vi "WLAN_SNR_LTF.vi"(11 "LTF Corrected":cdb[](array[numeric])) -> (0 "SNR Valid?":bool, 1 "Noise Power":dbl, 2 "Signal Power":dbl, 3 "SNR dB":dbl)   [LabVIEW 2022 SP3]
uses:
  <vilib>/Analysis/2dsp.llb/Complex FFT.vi
  <vilib>/Analysis/baseanly.llb/Mean (DBL).vi
  <vilib>/Analysis/NI_AALPro.lvlib
  <vilib>/Analysis/NI_AALBase.lvlib
panel:
  out "size(s) 4":i32
  out "size(s) 5":i32
  out "size(s) 3":i32
  out "size(s) 2":i32
  out "size(s)":i32
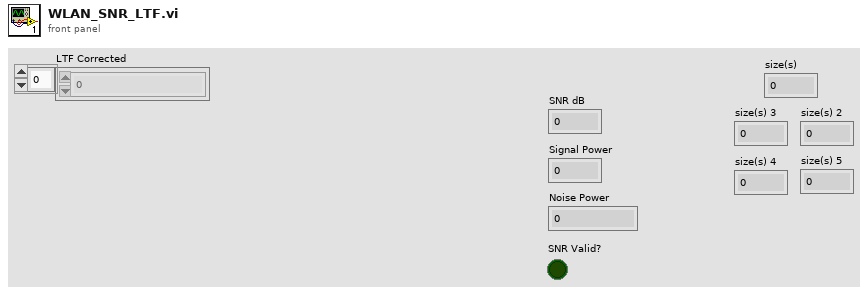
[diagram p1: front panel]
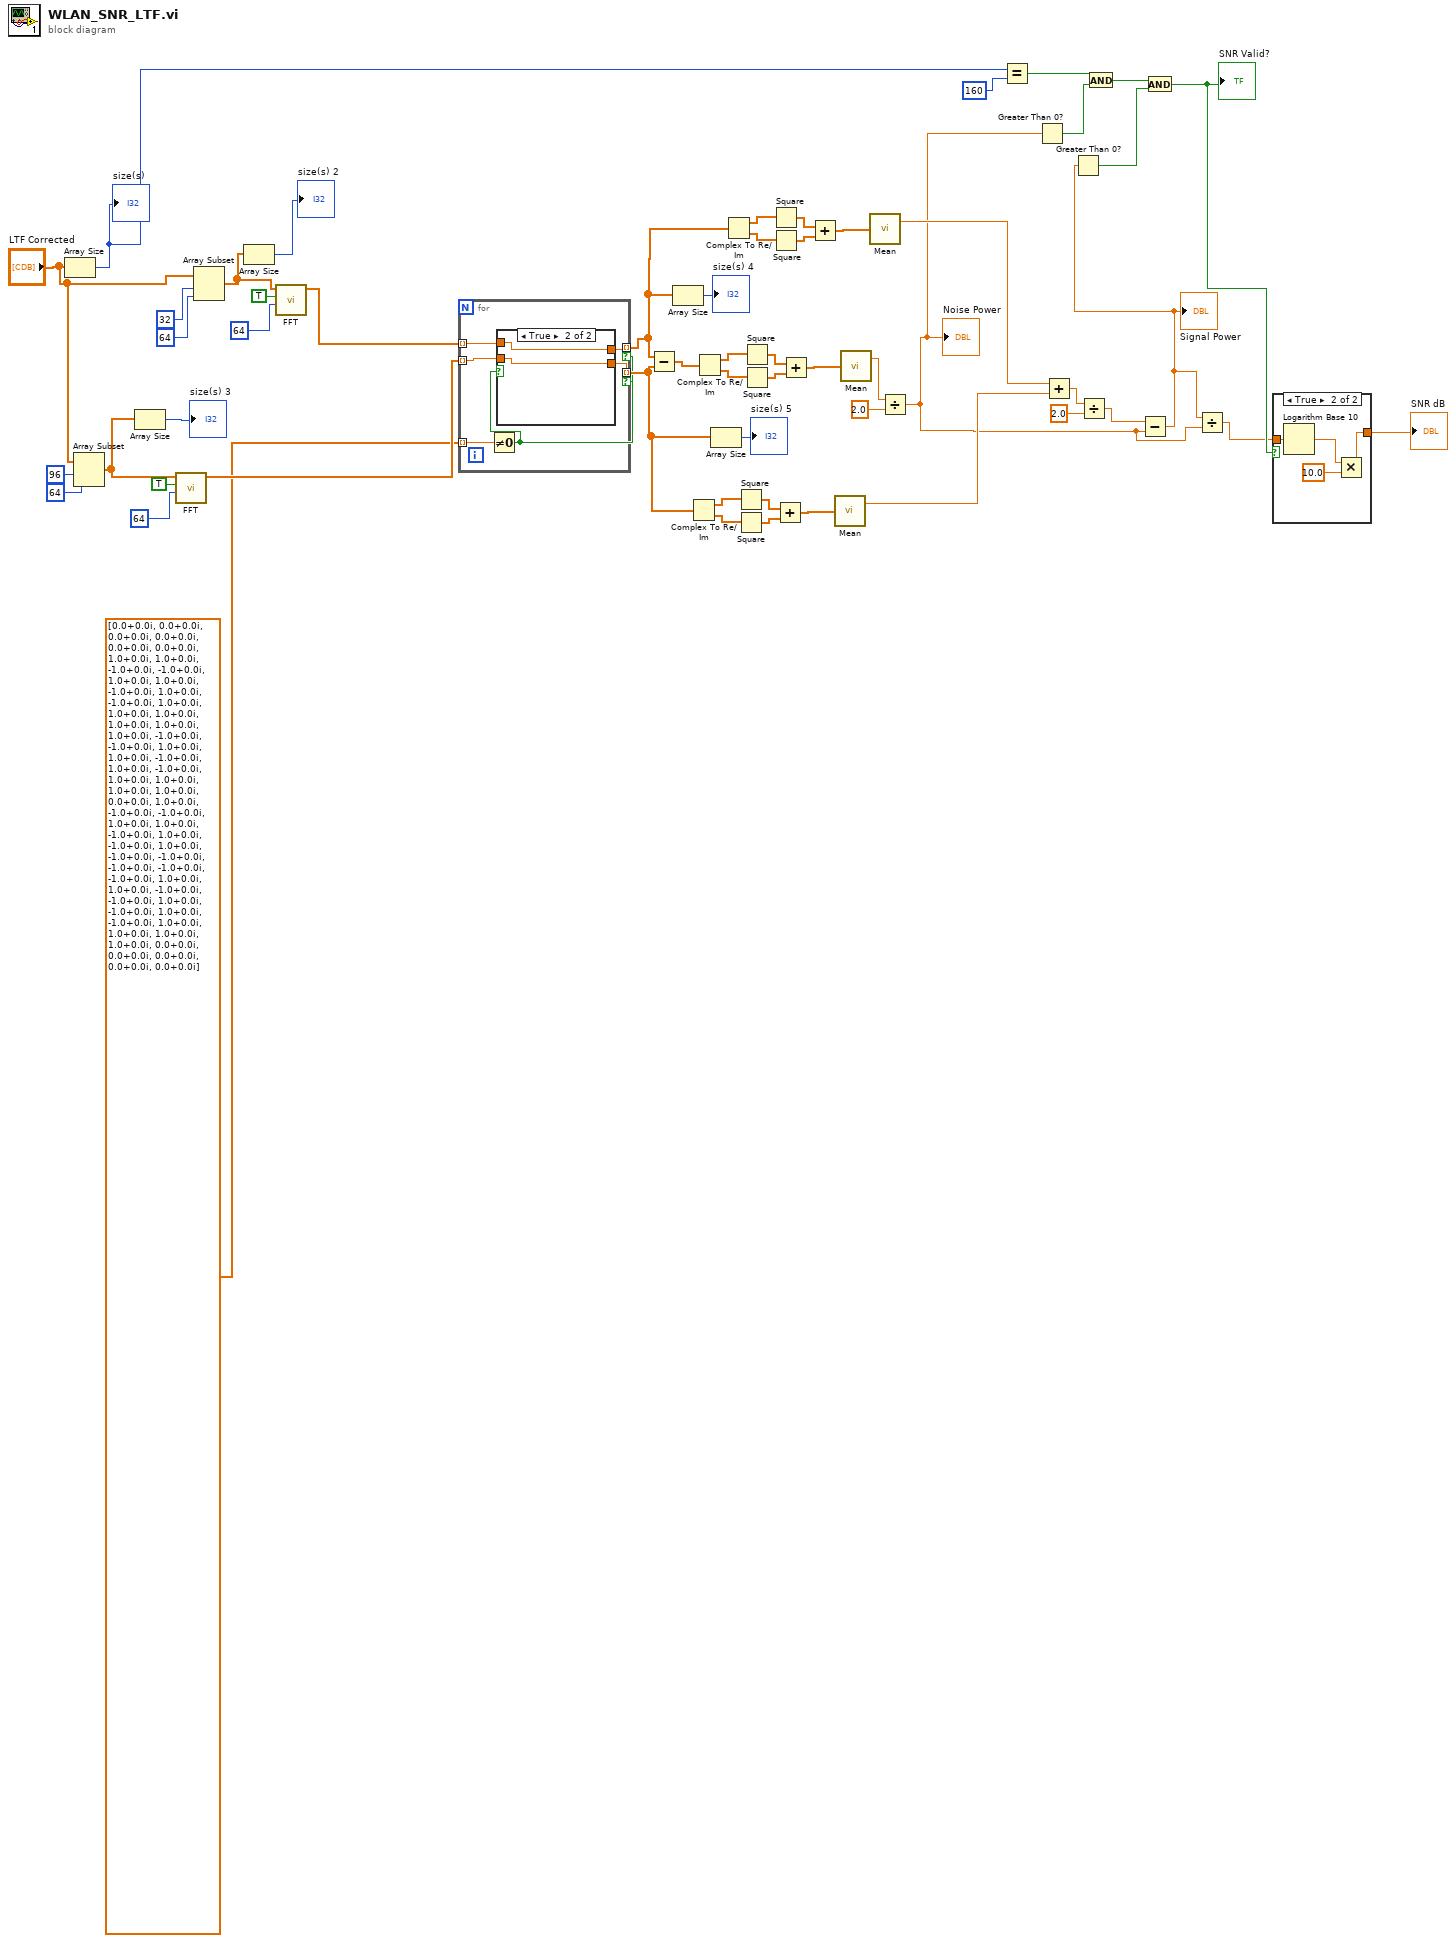
[diagram p0: block diagram]
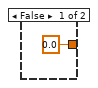
[diagram p2: hidden frame]
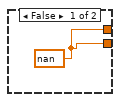
[diagram p3: hidden frame]
diagram:
  n1 = Array Size(array="LTF Corrected") -> (size(s)=w11:i32)
  "size(s)" <- w11
  n2 = Array Subset(array="LTF Corrected", index=96, length=64) -> (w42:cdb[])
  n3 = Array Size(array=w42) -> (size(s)=→"size(s) 3":i32)
  n4 = call-poly <vilib>:"FFT.vi"("FFT size"=64, "shift?"=TRUE, "X"=w42) -> ("FFT {X}"=w40:cdb[])  [unwired: 7 in, 1 out]
  n5 = Array Subset(array="LTF Corrected", index=32, length=64) -> (w43:cdb[])
  n6 = Array Size(array=w43) -> (size(s)=→"size(s) 2":i32)
  n7 = call-poly <vilib>:"FFT.vi"("FFT size"=64, "shift?"=TRUE, "X"=w43) -> ("FFT {X}"=w41:cdb[])  [unwired: 7 in, 1 out]
  n8 = for {
    tunnel: w41 -> [w58] mode=indexing
    tunnel: w40 -> [w59] mode=indexing
    tunnel: cdb[] [0.0+0.0i, 0.0+0.0i, 0.0+0.0i, 0.0+0.0i, 0.0+0.0i, 0.0+0.0i, 1.0+0.0i, 1.0+0.0i, -1.0+0.0i, -1.0+0.0i, 1.0+0.0i, 1.0+0.0i, -1.0+0.0i, 1.0+0.0i, -1.0+0.0i, 1.0+0.0i, 1.0+0.0i, 1.0+0.0i, 1.0+0.0i, 1.0+0.0i, 1.0+0.0i, -1.0+0.0i, -1.0+0.0i, 1.0+0.0i, 1.0+0.0i, -1.0+0.0i, 1.0+0.0i, -1.0+0.0i, 1.0+0.0i, 1.0+0.0i, 1.0+0.0i, 1.0+0.0i, 0.0+0.0i, 1.0+0.0i, -1.0+0.0i, -1.0+0.0i, 1.0+0.0i, 1.0+0.0i, -1.0+0.0i, 1.0+0.0i, -1.0+0.0i, 1.0+0.0i, -1.0+0.0i, -1.0+0.0i, -1.0+0.0i, -1.0+0.0i, -1.0+0.0i, 1.0+0.0i, 1.0+0.0i, -1.0+0.0i, -1.0+0.0i, 1.0+0.0i, -1.0+0.0i, 1.0+0.0i, -1.0+0.0i, 1.0+0.0i, 1.0+0.0i, 1.0+0.0i, 1.0+0.0i, 0.0+0.0i, 0.0+0.0i, 0.0+0.0i, 0.0+0.0i, 0.0+0.0i] -> [w60] mode=indexing
    tunnel: [w57] -> w23 mode=indexing if=w55
    tunnel: [w56] -> w17 mode=indexing if=w55
    n9 = Not Equal To 0?(x=w60) -> (x != 0?=w55:bool)
    n10 = case shown="True" w55 {
      tunnel: w59 -> [_ w62]
      tunnel: w58 -> [_ w63]
      tunnel: [w61 w63] -> w57
      tunnel: [w61 w62] -> w56
      frame False {
        w61 = nan
      }
      frame True {
      }
    }
  }
  n11 = Subtract(x=w23, y=w17) -> (x-y=w36:cdb[])
  n12 = Array Size(array=w23) -> (size(s)=→"size(s) 4":i32)
  n13 = Complex To Re/Im(x + iy=w17) -> (x=w22:dbl[], y=w21:dbl[])
  n14 = Complex To Re/Im(x + iy=w36) -> (x=w35:dbl[], y=w34:dbl[])
  n15 = Array Size(array=w17) -> (size(s)=→"size(s) 5":i32)
  n16 = Complex To Re/Im(x + iy=w23) -> (x=w28:dbl[], y=w27:dbl[])
  n17 = Square(x=w22) -> (x^2=w20:dbl[])
  n18 = Square(x=w21) -> (x^2=w19:dbl[])
  n19 = Square(x=w35) -> (x^2=w33:dbl[])
  n20 = Square(x=w34) -> (x^2=w32:dbl[])
  n21 = Square(x=w28) -> (x^2=w26:dbl[])
  n22 = Square(x=w27) -> (x^2=w25:dbl[])
  n23 = Add(x=w20, y=w19) -> (x+y=w18:dbl[])
  n24 = Add(x=w33, y=w32) -> (x+y=w31:dbl[])
  n25 = Add(x=w26, y=w25) -> (x+y=w24:dbl[])
  n26 = call-poly <vilib>:"Mean.vi"("X"=w18) -> ("mean"=w15:dbl)  [unwired: 1 out]
  n27 = call-poly <vilib>:"Mean.vi"("X"=w31) -> ("mean"=w30:dbl)  [unwired: 1 out]
  n28 = call-poly <vilib>:"Mean.vi"("X"=w24) -> ("mean"=w16:dbl)  [unwired: 1 out]
  n29 = Divide(x=w30, y=2.0) -> (x/y=w9:dbl)
  "Noise Power" <- w9
  n30 = Equal?(x=w11, y=160) -> (x = y?=w7:bool)
  n31 = Greater Than 0?(x=w9) -> (x > 0?=w6:bool)
  n32 = Add(x=w16, y=w15) -> (x+y=w13:dbl)
  n33 = Divide(x=w13, y=2.0) -> (x/y=w12:dbl)
  n34 = And(x=w7, y=w6) -> (x .and. y?=w4:bool)
  n35 = Subtract(x=w12, y=w9) -> (x-y=w8:dbl)
  "Signal Power" <- w8
  n36 = Greater Than 0?(x=w8) -> (x > 0?=w5:bool)
  n37 = And(x=w4, y=w5) -> (x .and. y?=w3:bool)
  "SNR Valid?" <- w3
  n38 = Divide(x=w8, y=w9) -> (x/y=w1:dbl)
  n39 = case shown="True" w3 {
    tunnel: [0.0 w65] -> w2
    tunnel: w1 -> [_ w66]
    frame False {
    }
    frame True {
      n40 = Logarithm Base 10(1:w66) -> (0:w68:dbl)
      n41 = Multiply(x=w68, y=10.0) -> (x*y=w65:dbl)
    }
  }
  "SNR dB" <- w2
